vi "Find or Add List Item.vi"(7 "Name":string, 8 "error in":errorcluster, 9 "ID":string, 10 "IDs":string[](array[string]), 11 "Names":string[](array[string])) -> (0 "error out":errorcluster, 1 "Index":i32, 2 "IDs out":string[](array[string]), 3 "Names out":string[](array[string]))   [LabVIEW 2026]
doc: "Finds ID in IDs and returns its index, for selecting an item in a ring whose items are Names (Names and IDs are parallel).\n\nIf ID is not empty and not in IDs, Name and ID are appended to the lists and Index is the new last item - so an entry whose project or task has since been made inactive still shows it. If ID is empty, the lists are unchanged and Index is 0.\n\nError in passes through unchanged.\n\nInputs: Names; IDs; ID; Name (shown when ID has to be added); error in.\nOutputs: Names out; IDs out; Index; error out.\n\nGenerated by: Claude"
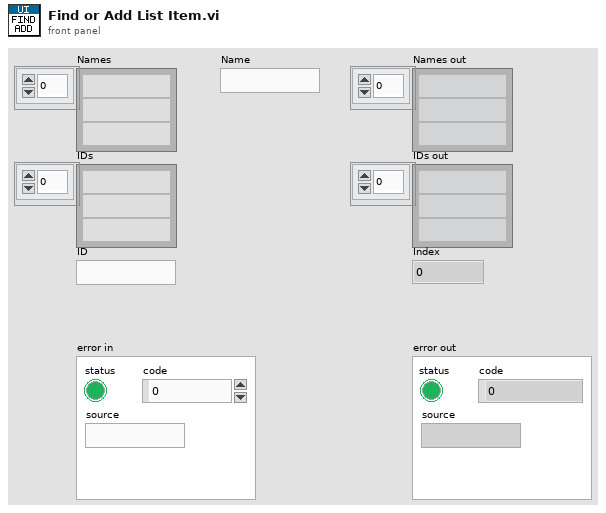
[diagram p1: front panel]
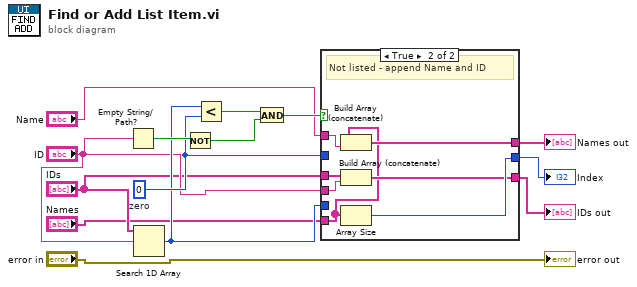
[diagram p0: block diagram]
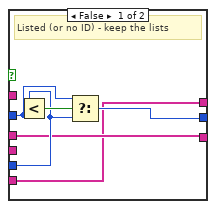
[diagram p2: hidden frame]
diagram:
  w10 = 0  # zero
  n1 = Empty String/Path?(string/path="ID") -> (empty?=w12:bool)
  n2 = Search 1D Array(1D array="IDs", element="ID") -> (index of element=w9:i32)  [unwired: 1 in]
  n3 = Not(x=w12) -> (.not. x?=w13:bool)
  n4 = Less?(x=w9, y=w10) -> (x < y?=w11:bool)
  n5 = And(x=w11, y=w13) -> (x .and. y?=w14:bool)
  n6 = case shown="True" w14 {
    tunnel: "Names" -> [w15 w21]
    tunnel: "IDs" -> [w16 w22]
    tunnel: "ID" -> [_ w23]
    tunnel: "Name" -> [_ w24]
    tunnel: w10 -> [w18 _]
    tunnel: w9 -> [w17 _]
    tunnel: [w15 w25] -> w6
    tunnel: [w16 w26] -> w7
    tunnel: [w20 w27] -> w8
    frame False {
      # "Listed (or no ID) - keep the lists"
      n7 = Less?(x=w17, y=w18) -> (x < y?=w19:bool)
      n8 = Select(t=w18, s=w19, f=w17) -> (s? t:f=w20:i32)
    }
    frame True {
      # "Not listed - append Name and ID"
      n9 = Build Array (concatenate)(w21, w24) -> (w25:string[])
      n10 = Build Array (concatenate)(w22, w23) -> (w26:string[])
      n11 = Array Size(array=w21) -> (size(s)=w27:i32)
    }
  }
  "Names out" <- w6
  "IDs out" <- w7
  "Index" <- w8
  "error out" <- "error in"
